vi "Set Group Scalar Channel Data.vi"(6 "error in (no error)":errorcluster, 7 "scalar channel in":T2 {"Data Type" format="%.0x"}, 9 "item ref in":T1 format="%.0x") -> (0 "error out":errorcluster, 3 "scalar channels out":T4[](array[typedef]) {"Item Ref" format="%.0x"})   [LabVIEW 2020, in "FPGA Addon System Explorer.lvlib"]
uses:
  FPGA Addon System Explorer.lvlib
  Types/Output Scalar.ctl
  Addon Shared/Types/FPGA Addon Data Type.ctl
  <vilib>/NI VeriStand/Custom Device API/Custom Device Item Ref.ctl
  Addon Shared/Types/Register Information.ctl
  Addon Shared/FPGA Addon Shared.lvlib
  <vilib>/NI VeriStand/Custom Device API/Custom Device API.lvlib
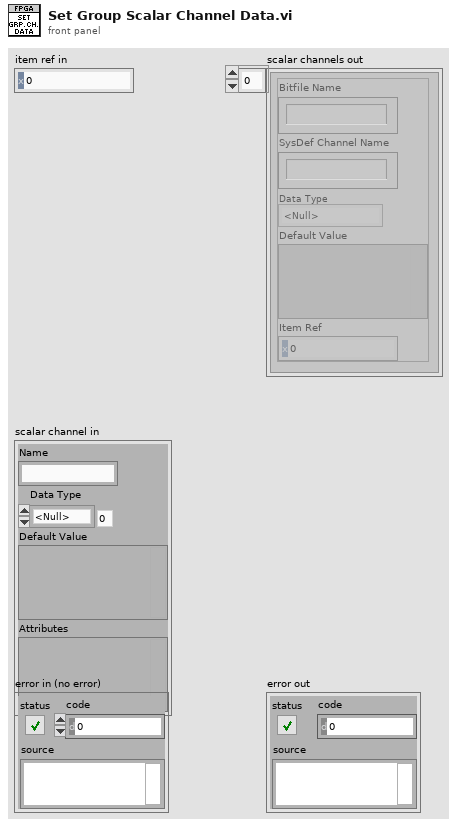
[diagram p1: front panel]
types:
  T1 = typedef "Custom Device API.lvlib/Custom Device Item Ref.ctl" = u64
  T2 = typedef "FPGA Addon Shared.lvlib/Register Information.ctl" = cluster{"Name":string, "Data Type":T3, "Default Value":variant, "Attributes":variant}
  T3 = typedef "FPGA Addon Shared.lvlib/FPGA Addon Data Type.ctl" = enum8{"<Null>", "I8", "I16", "I32", "I64", "U8", "U16", "U32", "U64", "SGL", "Boolean", "Analog PWM In Settings", "Analog PWM In", "Digital PWM In Settings", "Digital PWM In", "Digital PWM Out", "Sine Out", "FXP", "FXP+/-24.5", "FXP+/-16.5", "FXP+/-32.8", "FXP+/-64.32", "FXP+/-16.7", "FXP+/-20.5", "FXP+/-27.5", "FXP+/-32.16", "FXP+16.3", "FXP+18.3", "Digital Static In", "Digital Static Out", "Digital Static In Settings", "Digital WSS Out", "Quad Encoder Settings", "Quad Encoder In", "Group"}
  T4 = typedef "FPGA Addon System Explorer.lvlib/Output Scalar.ctl" = cluster{"Bitfile Name":string, "SysDef Channel Name":string, "Data Type":T3, "Default Value":variant, "Item Ref":T1}
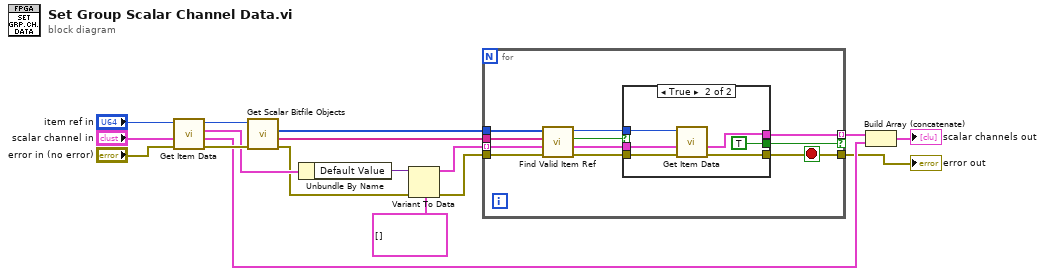
[diagram p0: block diagram]
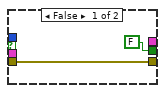
[diagram p2: hidden frame]
diagram:
  n1 = call "Get Item Data.vi"("error in (no error)"="error in (no error)", "scalar channel in"="scalar channel in", "item ref in"="item ref in") -> ("error out"=w16:errorcluster, "scalar channel data out"=w15:T4, "scalar channel out"=w7:T2, "item ref out"=w9:T1)  [unwired: 5 in]
  n2 = call "Get Scalar Bitfile Objects.vi"("error in"=w16, "item ref in"=w9) -> ("error out"=w2:errorcluster, "bitfile object names"=w12:string[], "section children refs"=w10:T1[])  [unwired: 6 in, 1 out]
  n3 = Unbundle By Name(w7) -> ("Default Value"=w8:variant)
  n4 = Variant To Data(error in=w2, type=T2[] [], Variant=w8) -> (data=w11:T2[], error out=w1:errorcluster)
  n5 = for {
    tunnel: w10 -> [w25]
    tunnel: w11 -> [w23] mode=indexing
    tunnel: w12 -> [w24]
    tunnel: w1 -> [w22]
    tunnel: [w26] -> w13
    tunnel: [w28] -> w14 mode=indexing if=w27
    stop <- w26 stop-if-true
    n6 = call "Find Valid Item Ref.vi"("error in (no error)"=w22, "scalar channels"=w23, "bitfile object names"=w24, "section children refs"=w25) -> ("error out"=w21:errorcluster, "scalar channel out"=w18:T2, "found"=w20:bool, "item ref out"=w19:T1)  [unwired: 4 in]
    n7 = case shown="True" w20 {
      tunnel: w21 -> [w29 w36]
      tunnel: [w29 w35] -> w26
      tunnel: [_ w34] -> w28
      tunnel: [FALSE TRUE] -> w27
      tunnel: w19 -> [_ w32]
      tunnel: w18 -> [_ w31]
      frame False {
      }
      frame True {
        n8 = call "Get Item Data.vi"("error in (no error)"=w36, "scalar channel in"=w31, "item ref in"=w32) -> ("error out"=w35:errorcluster, "scalar channel data out"=w34:T4)  [unwired: 5 in, 2 out]
      }
    }
  }
  "error out" <- w13
  n9 = Build Array (concatenate)(w14, w15) -> (→"scalar channels out":T4[])
